vi "Get array of String.vi"(8 "error in (no error)":errorcluster, 10 "Name":string, 11 "json class in":refnum<class "json class.lvclass">) -> (0 "error out":errorcluster, 2 "String Array":string[](array[string]), 3 "json class out":refnum<class "json class.lvclass">)   [LabVIEW 2021, in "Config Library.lvlib" / "json class.lvclass"]
uses:
  json class.lvclass
  json class.lvclass/json class.ctl
  <vilib>/addons/JSON API/JSON Scalar/JSON Scalar.lvclass
  <vilib>/addons/JSON API/JSON Array/JSON Array.lvclass
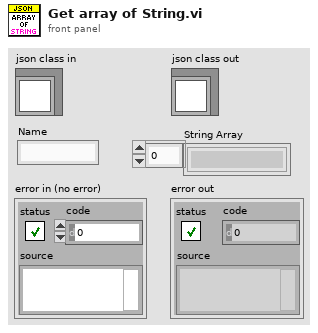
[diagram p1: front panel]
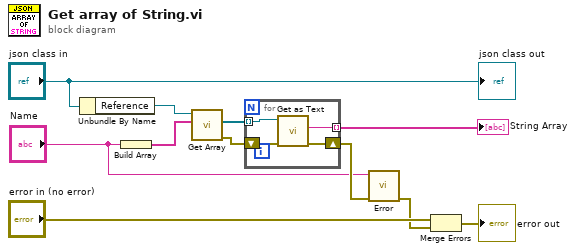
[diagram p0: block diagram]
diagram:
  n1 = Unbundle By Name("json class in") -> ("Reference"=w7:refnum<class "JSON Value.lvclass">)
  n2 = Build Array("Name") -> (w6:string[])
  n3 = call <vilib>:"Get Array.vi"("Name Array"=w6, "JSON Array in"=w7) -> ("error out"=w4:errorcluster, "Array"=w5:refnum<class "JSON Value.lvclass">[])  [unwired: 7 in, 1 out]
  n4 = for {
    tunnel: [w14] -> w8 mode=indexing
    tunnel: w5 -> [w13] mode=indexing
    shift-right: [w15] -> w3
    shift-left: w4 -> [w12]
    n5 = call <vilib>:"Get as Text.vi"("error in (no error)"=w12, "JSON Scalar in"=w13) -> ("error out"=w15:errorcluster, "LabVIEW Text"=w14:string)  [unwired: 7 in, 1 out]
  }
  "String Array" <- w8
  n6 = call "Error.vi"("error in (no error)"=w3, "Name"="Name") -> ("error out"=w1:errorcluster)  [unwired: 9 in]
  n7 = Merge Errors("error in (no error)", w1) -> (→"error out":errorcluster)
  "json class out" <- "json class in"
